vi "Lab_5_Calculate_HR_Zones.vi"(8 "error in":errorcluster, 11 "HD Data Structure":T1) -> (0 "error out":errorcluster, 3 "HD Data Structure":T1)   [LabVIEW 2025]
uses:
  Lab 3/Control og.ctl
  Lab 3/Control Runners.ctl
  Lab 3/Control Raw.ctl
  <vilib>/Analysis/baseanly.llb/Mean (DBL).vi
  <vilib>/Analysis/NI_AALBase.lvlib
panel:
  out "XY Graph":cluster{dbl[], "Heart Rate Zone No":dbl[]}(graph)
  out "BPM":cluster{"Time":timestamp[], "Bpm":i32[]}(graph)
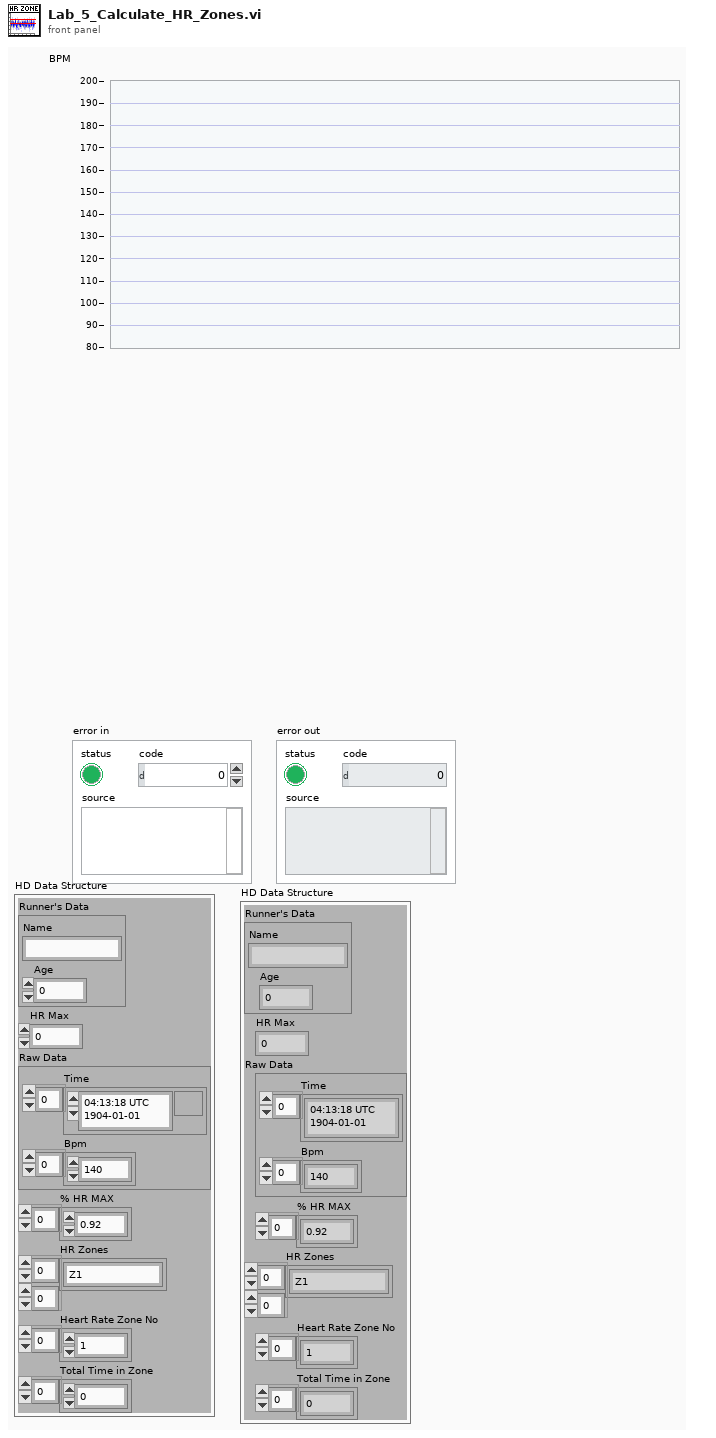
[diagram p1: front panel]
types:
  T1 = typedef "Control og.ctl" = cluster{"Runner's Data":T2, "HR Max":i32, "Raw Data":T3, "% HR MAX ":dbl[], "HR Zones":string[][], "Heart Rate Zone No":dbl[], "Total Time in Zone":dbl[]}
  T2 = typedef "Control Runners.ctl" = cluster{"Name":string, "Age":i32}
  T3 = typedef "Control Raw.ctl" = cluster{"Time":timestamp[], "Bpm":i32[]}
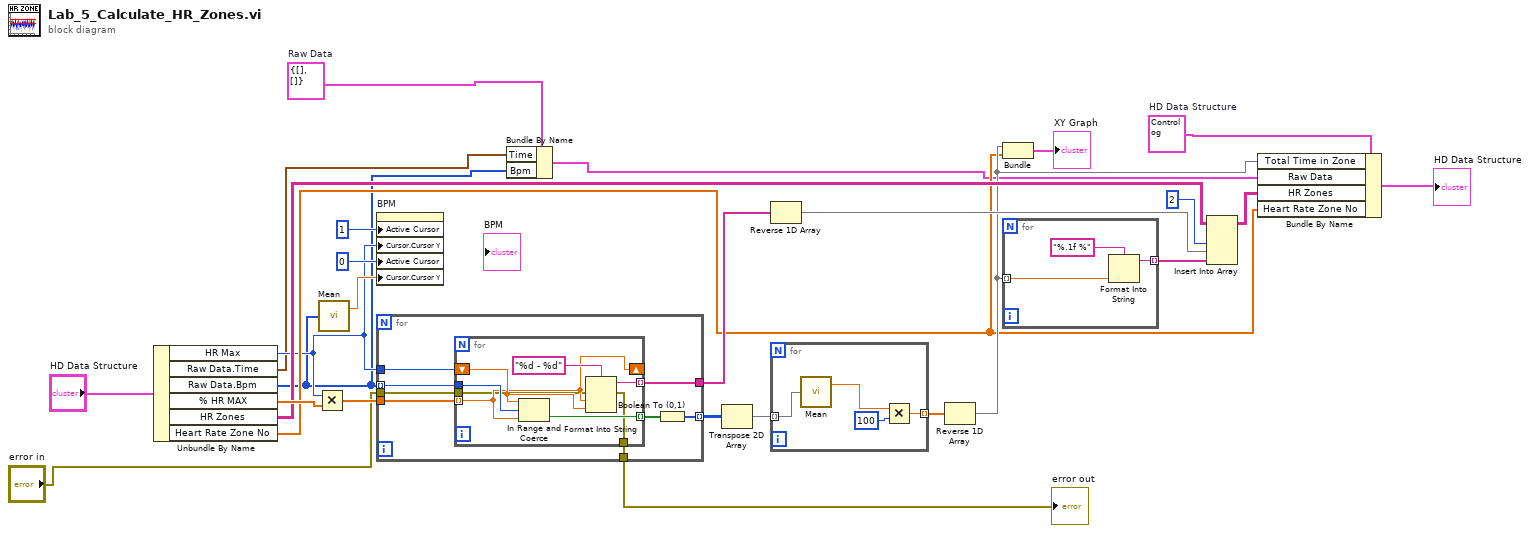
[diagram p0: block diagram]
diagram:
  w4 = T1 data[18182B]  # HD Data Structure
  w5 = T3 {"Time"=[], "Bpm"=[]}  # Raw Data
  n1 = Unbundle By Name("HD Data Structure") -> ("HR Max"=w12:i32, "Raw Data.Time"=w9:timestamp[], "Raw Data.Bpm"=w8:i32[], "% HR MAX"=w17:dbl[], "HR Zones"=w16:string[][], "Heart Rate Zone No"=w13:dbl[])
  n2 = Multiply(x=w12, y=w17) -> (x*y=w27:dbl[])
  n3 = call-poly <vilib>:"Mean.vi"("X"=w8) -> ("mean"=w18:dbl)  [unwired: 1 out]
  n4 = property on="BPM" class="XYGraph (strict)"("Active Cursor"=1, "Cursor.Cursor Y"=w12, "Active Cursor"=0, "Cursor.Cursor Y"=w18) -> ()  [unwired: 2 in, 2 out]
  n5 = for {
    tunnel: w27 -> [w35]
    tunnel: w8 -> [w34] mode=indexing
    tunnel: [w33] -> w25
    tunnel: w12 -> [w32]
    tunnel: [w30] -> w2 mode=indexing
    tunnel: [w29] -> w11
    tunnel: "error in" -> [w28]
    n6 = for {
      shift-right: [w40] -> _
      shift-left: w32 -> [w41]
      tunnel: w35 -> [w40] mode=indexing
      tunnel: w34 -> [w42]
      tunnel: [w39] -> w33 mode=indexing
      tunnel: [w38] -> w31 mode=indexing
      tunnel: [w37] -> w29
      tunnel: w28 -> [w36]
      n7 = In Range and Coerce(upper limit=w41, x=w42, lower limit=w40) -> (In Range?=w38:bool)  [unwired: 1 out]
      n8 = Format Into String(format string="%d - %d", error in=w36, w40, w41) -> (resulting string=w39:string, error out=w37:errorcluster)  [unwired: 1 in]
    }
    n9 = Boolean To (0,1)(Boolean=w31) -> (0, 1=w30:i16[])
  }
  "error out" <- w11
  n10 = Bundle By Name(cluster=w5, "Time"=w9, "Bpm"=w8) -> (w7:T3)
  n11 = Transpose 2D Array(2D array=w2) -> (transposed array=w1:i16[][])
  n12 = Reverse 1D Array(array=w25) -> (reversed array=w24:string[])
  n13 = for {
    tunnel: w1 -> [w47] mode=indexing
    tunnel: [w45] -> w22 mode=indexing
    n14 = call-poly <vilib>:"Mean.vi"("X"=w47) -> ("mean"=w44:dbl)  [unwired: 1 out]
    n15 = Multiply(x=w44, y=100) -> (x*y=w45:dbl)
  }
  n16 = Reverse 1D Array(array=w22) -> (reversed array=w14:dbl[])
  n17 = Bundle(w14, "Heart Rate Zone No"=w13) -> (→"XY Graph":cluster{dbl[], "Heart Rate Zone No":dbl[]})  [unwired: 1 in]
  n18 = for {
    tunnel: w14 -> [w50] mode=indexing
    tunnel: [w48] -> w21 mode=indexing
    n19 = Format Into String(format string="%.1f %", w50) -> (resulting string=w48:string)  [unwired: 2 in, 1 out]
  }
  n20 = Insert Into Array(array=w16, index (col)=2, new element #1=w24, new element #2=w21) -> (w15:string[][])  [unwired: 1 in]
  n21 = Bundle By Name(cluster=w4, "Total Time in Zone"=w14, "Raw Data"=w7, "HR Zones"=w15, "Heart Rate Zone No"=w13) -> (→"HD Data Structure":T1)
